vi "STD recal.vi"(8 "Mx Level intensity":dbl, 9 "STD Type":enum16{"Region", "Each", "Fixed"}(ring), 10 "BR BL and STD info":T3, 11 "B Cluster":T1) -> (0 "SN [ratio]":T2, 3 "std [ratio]":T4)   [LabVIEW 2018]
panel:
  out "R S/N ratio":dbl
  out "B S/N ratio":dbl
  out "B std [pA]":dbl
  out "R std [ratio]":dbl
  out "B std [%]":dbl
  out "Mx Intensity Level [pA]":dbl
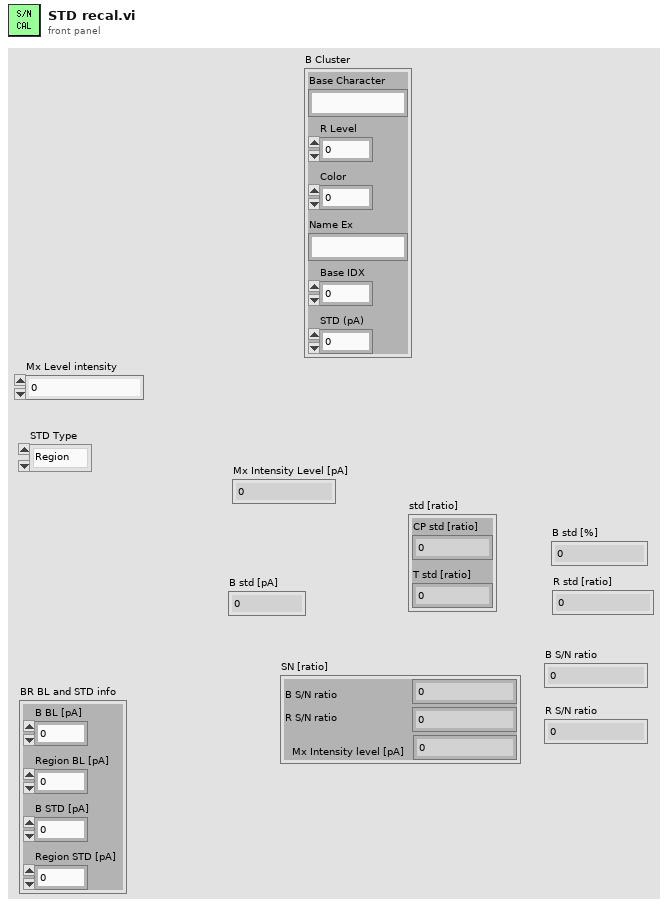
[diagram p1: front panel]
types:
  T1 = cluster{"Base Character":string, "R Level":dbl, "Color":u32, "Name Ex":string, "Base IDX":dbl, "STD (pA)":dbl}
  T2 = cluster{"B S/N ratio":dbl, "R S/N ratio":dbl, "Mx Intensity level [pA]":dbl}
  T3 = cluster{"B BL [pA]":dbl, "Region BL [pA]":dbl, "B STD [pA]":dbl, "Region STD [pA]":dbl}
  T4 = cluster{"CP std [ratio]":dbl, "T std [ratio]":dbl}
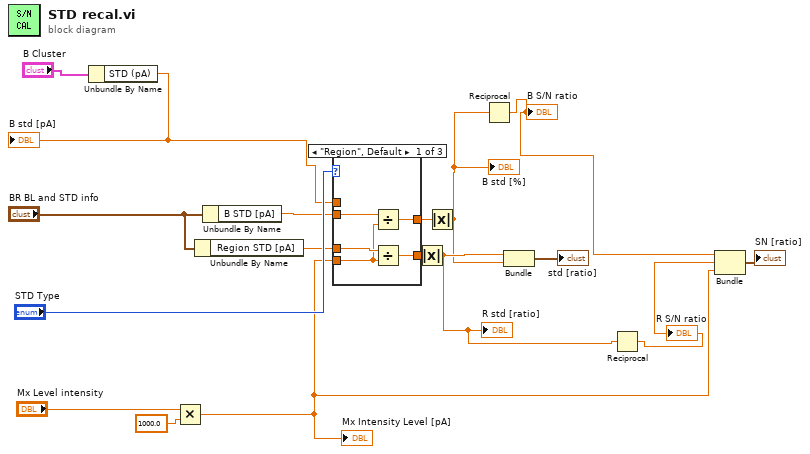
[diagram p0: block diagram]
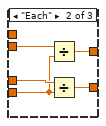
[diagram p2: hidden frame]
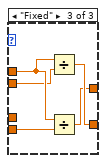
[diagram p3: hidden frame]
diagram:
  n1 = Unbundle By Name("B Cluster") -> ("STD (pA)"=w3:dbl)
  "B std [pA]" <- w3
  n2 = Multiply(x="Mx Level intensity", y=1000.0) -> (x*y=w5:dbl)
  "Mx Intensity Level [pA]" <- w5
  n3 = Unbundle By Name("BR BL and STD info") -> ("Region STD [pA]"=w13:dbl)
  n4 = Unbundle By Name("BR BL and STD info") -> ("B STD [pA]"=w11:dbl)
  n5 = case shown="\"Region\", Default" "STD Type" {
    tunnel: w13 -> [w22 w24 _]
    tunnel: w5 -> [w19 w23 w31]
    tunnel: [w21 w27 w32] -> w9
    tunnel: w11 -> [w20 w25 w28]
    tunnel: [w18 w26 w30] -> w10
    tunnel: w3 -> [_ _ w29]
    frame "Region", Default {
      n6 = Divide(x=w20, y=w19) -> (x/y=w18:dbl)
      n7 = Divide(x=w22, y=w19) -> (x/y=w21:dbl)
    }
    frame "Each" {
      n8 = Divide(x=w25, y=w23) -> (x/y=w26:dbl)
      n9 = Divide(x=w24, y=w23) -> (x/y=w27:dbl)
    }
    frame "Fixed" {
      n10 = Divide(x=w29, y=w28) -> (x/y=w32:dbl)
      n11 = Divide(x=w29, y=w31) -> (x/y=w30:dbl)
    }
  }
  n12 = Absolute Value(x=w9) -> (abs(x)=w2:dbl)
  "R std [ratio]" <- w2
  n13 = Absolute Value(x=w10) -> (abs(x)=w1:dbl)
  "B std [%]" <- w1
  n14 = Reciprocal(x=w1) -> (1/x=w7:dbl)
  "B S/N ratio" <- w7
  n15 = Bundle(w2, w1) -> (→"std [ratio]":cluster{dbl, dbl})  [unwired: 1 in]
  n16 = Reciprocal(x=w2) -> (1/x=w6:dbl)
  "R S/N ratio" <- w6
  n17 = Bundle(w7, w6, w5) -> (→"SN [ratio]":cluster{dbl, dbl, dbl})  [unwired: 1 in]
